vi "Parse Error XML.vi"(9 "Code Tag Value":string, 10 "Error XML":string, 11 "AWS Core":refnum<class "Queue.lvclass">) -> (1 "Error Description Override":string, 2 "Error Code":i32, 3 "Warning":bool)   [LabVIEW 2015, in "NI_AWS_SQS.lvlib" / "Queue.lvclass"]
uses:
  Queue.lvclass
  Core/HTTP Request/HTTP Request.lvclass
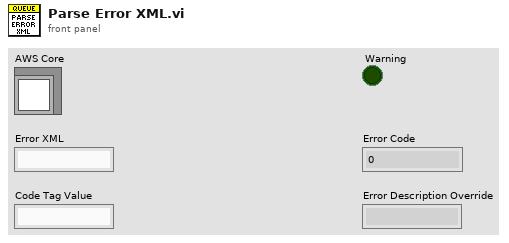
[diagram p1: front panel]
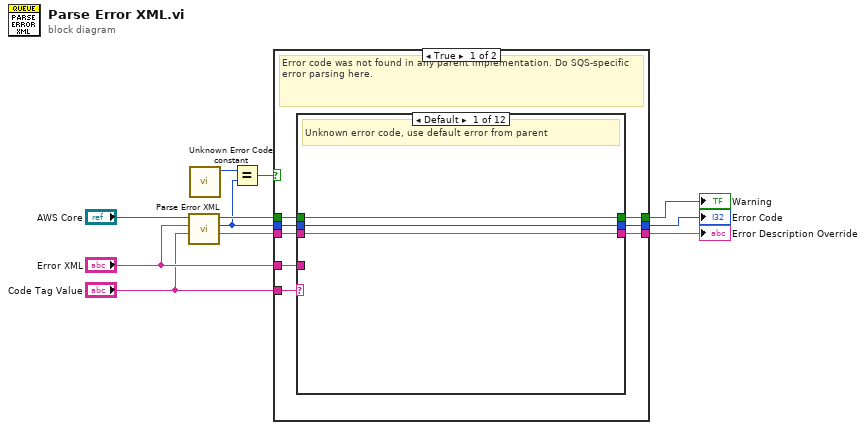
[diagram p0: block diagram]
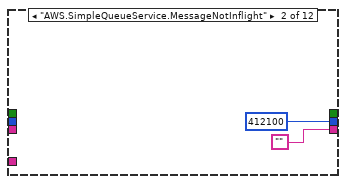
[diagram p2: hidden frame]
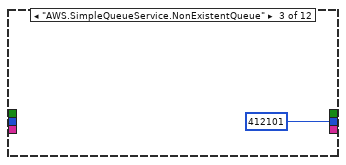
[diagram p3: hidden frame]
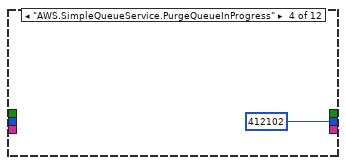
[diagram p4: hidden frame]
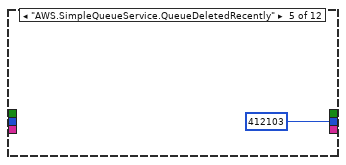
[diagram p5: hidden frame]
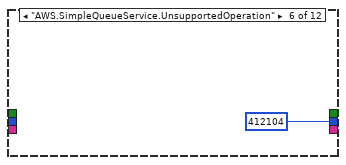
[diagram p6: hidden frame]
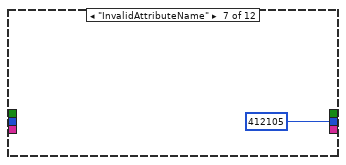
[diagram p7: hidden frame]
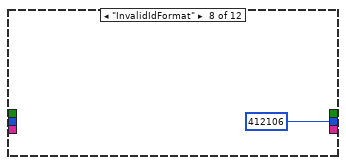
[diagram p8: hidden frame]
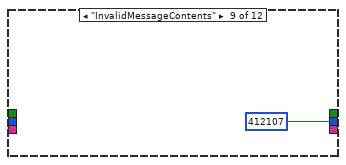
[diagram p9: hidden frame]
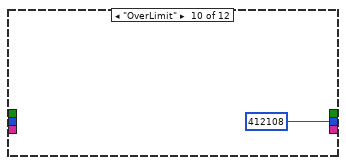
[diagram p10: hidden frame]
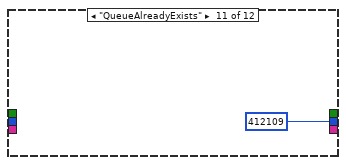
[diagram p11: hidden frame]
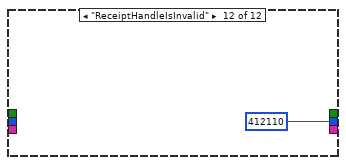
[diagram p12: hidden frame]
diagram:
  n1 = call-parent "Parse Error XML.vi"("Code Tag Value"="Code Tag Value", "Error XML"="Error XML", "AWS Core"="AWS Core") -> ("Error Description Override"=w9:string, "Error Code"=w1:i32, "Warning"=w10:bool)  [unwired: 6 in]
  n2 = call "Unknown Error Code constant.vi"() -> ("AWS Unknown Error Code value"=w3:i32)  [unwired: 11 in]
  n3 = Equal?(x=w3, y=w1) -> (x = y?=w2:bool)
  n4 = case shown="True" w2 {
    tunnel: w10 -> [w17 w37]
    tunnel: w9 -> [w15 w36]
    tunnel: [w14 w37] -> w8
    tunnel: [w12 w36] -> w7
    tunnel: [w13 w35] -> w6
    tunnel: "Error XML" -> [w19 _]
    tunnel: "Code Tag Value" -> [w18 _]
    tunnel: w1 -> [w16 w35]
    frame True {
      # "Error code was not found in any parent implementation. Do SQS-specific error parsing here."
      n5 = case shown="Default" w18 {
        tunnel: w19 -> [_ _ _ _ _ _ _ _ _ _ _ _]
        tunnel: w17 -> [w22 _ _ _ _ _ _ _ _ _ _ _]
        tunnel: w16 -> [w21 _ _ _ _ _ _ _ _ _ _ _]
        tunnel: w15 -> [w20 _ _ _ _ _ _ _ _ _ _ _]
        tunnel: [w22 _ _ _ _ _ _ _ _ _ _ _] -> w14
        tunnel: [w21 412100 412101 412102 412103 412104 412105 412106 412107 412108 412109 412110] -> w13
        tunnel: [w20 "" _ _ _ _ _ _ _ _ _ _] -> w12
        frame Default {
          # "Unknown error code, use default error from parent"
        }
        frame "AWS.SimpleQueueService.MessageNotInflight" {
        }
        frame "AWS.SimpleQueueService.NonExistentQueue" {
        }
        frame "AWS.SimpleQueueService.PurgeQueueInProgress" {
        }
        frame "AWS.SimpleQueueService.QueueDeletedRecently" {
        }
        frame "AWS.SimpleQueueService.UnsupportedOperation" {
        }
        frame "InvalidAttributeName" {
        }
        frame "InvalidIdFormat" {
        }
        frame "InvalidMessageContents" {
        }
        frame "OverLimit" {
        }
        frame "QueueAlreadyExists" {
        }
        frame "ReceiptHandleIsInvalid" {
        }
      }
    }
    frame False {
      # "Parent method already assigned an error code"
    }
  }
  "Error Description Override" <- w7
  "Warning" <- w8
  "Error Code" <- w6
